vi "Config.vi"(8 "error in (no error)":errorcluster, 10 "Setting":variant, 11 "KE65XX DMM in":refnum<class "Keithley 65XX DMM.lvclass">) -> (0 "error out":errorcluster, 3 "KE65XX DMM out":refnum<class "Keithley 65XX DMM.lvclass">)   [LabVIEW 2025, in "DMM.lvlib" / "Keithley 65XX DMM.lvclass"]
uses:
  Keithley 65XX DMM.lvclass
  C:/Users/Public/Documents/Sandia National Labs/TSS Plugin/CEF.lvlibp/Node/CEF_Node.lvclass
  C:/Working copy/TS Manager/Plugin/Engines/DMM/DMM Instrument/DMM Instrument.lvclass
  C:/Users/Public/Documents/Sandia National Labs/TSS Plugin/Abstract Engine.lvlibp/Abstract Instrument/Abstract Instrument.lvclass
  DMM configuration/DMM configuration.lvclass
  Keithley 65XX DMM.lvclass/Keithley 65XX DMM.ctl
  DMM configuration/DMM configuration.lvclass/DMM configuration.ctl
  DMM Channel/DMM Channel.lvclass
  Users/Public/Documents/Sandia National Labs/TSS Plugin/Abstract Engine.lvlibp/Abstract Instrument/Channel.ctl
  Users/Public/Documents/Sandia National Labs/TSS Plugin/Abstract Engine.lvlibp/Abstract Instrument/Data Type.ctl
  Users/Public/Documents/Sandia National Labs/TSS Plugin/Abstract Engine.lvlibp/Channel configuration/Channel configuration.lvclass
  DMM configuration/Read DMM Setting.vi
  Users/Public/Documents/Sandia National Labs/TSS Plugin/CEF.lvlibp/Node/ReadChildren.vi
  Users/Public/Documents/Sandia National Labs/TSS Plugin/Abstract Engine.lvlibp/Channel configuration/Read Channel Setting.vi
  Users/Public/Documents/Sandia National Labs/TSS Plugin/CEF.lvlibp/Node/CEF_Node.lvclass
  Users/Public/Documents/Sandia National Labs/TSS Plugin/CEF.lvlibp/serializable configuration/CEF_serializable configuration.lvclass
  <instrlib>/Keithley DMM6500 DAQ6500 Series/Keithley DMM6500 DAQ6500 Series.lvlib
  Users/Public/Documents/Sandia National Labs/TSS Plugin/Abstract Engine.lvlibp/Abstract Instrument/Abstract Instrument.lvclass
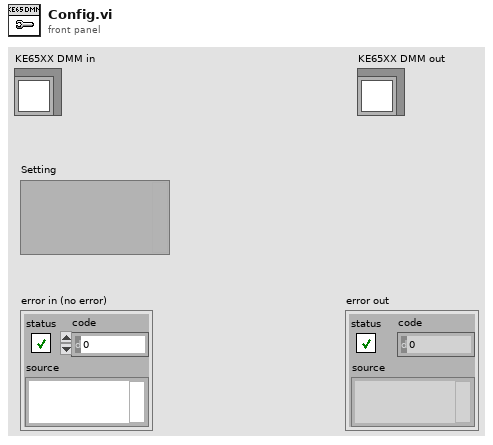
[diagram p1: front panel]
types:
  T1 = typedef "DMM.lvlib/DMM configuration.lvclass/DMM Setting.ctl" = cluster{"Function":string, "CurrentSource":string, "Resolution":string, "Range":dbl}
  T2 = typedef "Abstract Engine.lvlibp/Abstract Instrument.lvclass/Channel.ctl" = cluster{"Alias":string, "DataType":T3, "Unit":enum16{"---", "V", "A", "Ohm", "Hz", "uF", "degC", "deg"}, "Upper limit":dbl, "Lower limit":dbl, "Measurement":variant}
  T3 = typedef "Abstract Engine.lvlibp/Abstract Instrument.lvclass/Data Type.ctl" = string
  T4 = typedef "Abstract Engine.lvlibp/Channel configuration.lvclass/Default Channel.ctl" = cluster{"Address":string, "SW Alias":string, "Enabled":bool, "Type":string, "Description":string}
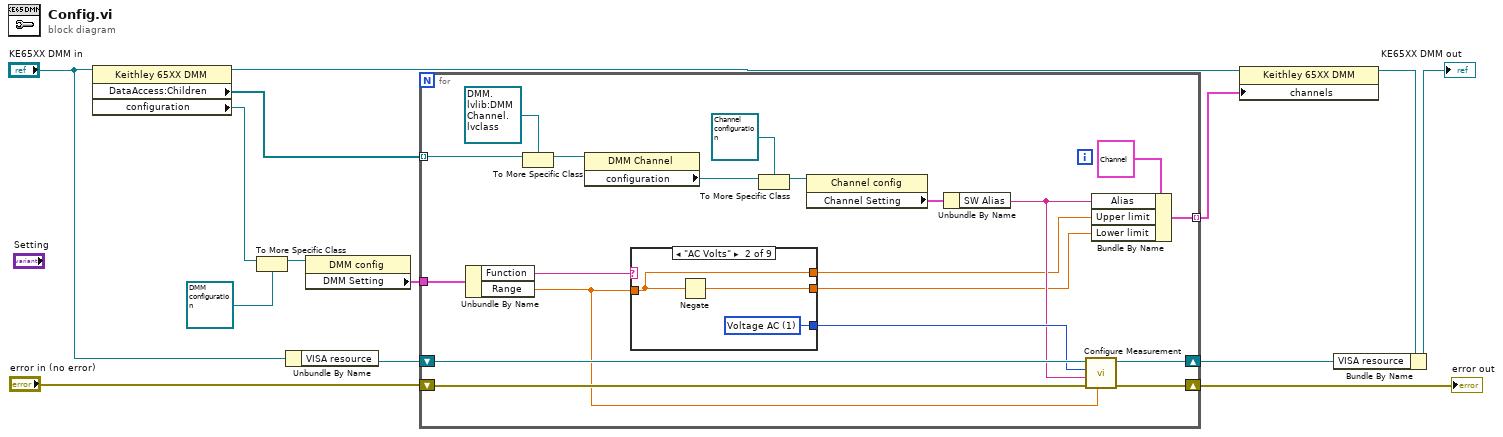
[diagram p0: block diagram]
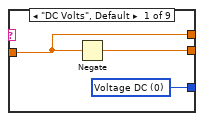
[diagram p2: hidden frame]
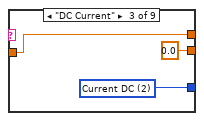
[diagram p3: hidden frame]
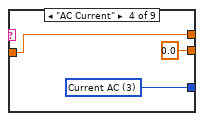
[diagram p4: hidden frame]
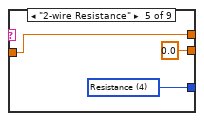
[diagram p5: hidden frame]
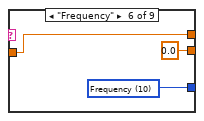
[diagram p6: hidden frame]
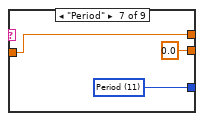
[diagram p7: hidden frame]
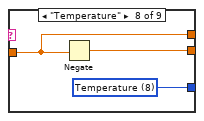
[diagram p8: hidden frame]
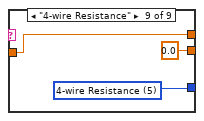
[diagram p9: hidden frame]
diagram:
  n1 = property class="Keithley 65XX DMM"(reference="KE65XX DMM in") -> (reference out=w11:refnum<class "Keithley 65XX DMM.lvclass">, "DataAccess:Children"=w8:refnum<data-value>[], "configuration"=w9:refnum<class "CEF_serializable configuration.lvclass">)  [unwired: 1 in, 1 out]
  n2 = To More Specific Class(target class=refnum<class "DMM configuration.lvclass"> refnum ("DMM.lvlib:DMM configuration.lvclass"), reference=w9) -> (specific class reference=w10:refnum<class "DMM configuration.lvclass">)  [unwired: 1 in, 1 out]
  n3 = Unbundle By Name("KE65XX DMM in") -> ("VISA resource"=w14:refnum<visa-resource-name>)
  n4 = property class="DMM config"(reference=w10) -> ("DMM Setting"=w5:T1)  [unwired: 1 in, 2 out]
  n5 = for {
    tunnel: w5 -> [w32]
    shift-right: [w33] -> w12
    shift-left: w14 -> [w34]
    tunnel: w8 -> [w29] mode=indexing
    shift-right: [w28] -> w7
    shift-left: "error in (no error)" -> [w27]
    tunnel: [w25] -> w1 mode=indexing
    n6 = Unbundle By Name(w32) -> ("Function"=w31:string, "Range"=w23:dbl)
    n7 = To More Specific Class(target class=refnum<data-value> refnum ("data value reference"), reference=w29) -> (specific class reference=w15:refnum<data-value>)  [unwired: 1 in, 1 out]
    n8 = property class="DMM Channel"(reference=w15) -> ("configuration"=w19:refnum<class "CEF_serializable configuration.lvclass">)  [unwired: 1 in, 2 out]
    n9 = case shown="\"AC Volts\"" w31 {
      tunnel: [w37 w40 w43 w46 w49 w52 w55 w58 w61] -> w30
      tunnel: w23 -> [w36 w39 w42 w45 w48 w51 w54 w57 w60]
      tunnel: [w36 w39 w42 w45 w48 w51 w54 w57 w60] -> w22
      tunnel: [w35 w38 0.0 0.0 0.0 0.0 0.0 w56 0.0] -> w21
      frame "DC Volts", Default {
        w37 = 0 items=[" Voltage DC", "Voltage AC", "Current DC", "Current AC", "Resistance", "4-wire Resistance", "Diode", "Capacitance", "Temperature", "Continuity", "Frequency", "Period", "Voltage Ratio"] ("Function (0: Voltage DC)")
        n10 = Negate(x=w36) -> (-x=w35:dbl)
      }
      frame "AC Volts" {
        w40 = 1 items=[" Voltage DC", "Voltage AC", "Current DC", "Current AC", "Resistance", "4-wire Resistance", "Diode", "Capacitance", "Temperature", "Continuity", "Frequency", "Period", "Voltage Ratio"] ("Function (0: Voltage DC)")
        n11 = Negate(x=w39) -> (-x=w38:dbl)
      }
      frame "DC Current" {
        w43 = 2 items=[" Voltage DC", "Voltage AC", "Current DC", "Current AC", "Resistance", "4-wire Resistance", "Diode", "Capacitance", "Temperature", "Continuity", "Frequency", "Period", "Voltage Ratio"] ("Function (0: Voltage DC)")
      }
      frame "AC Current" {
        w46 = 3 items=[" Voltage DC", "Voltage AC", "Current DC", "Current AC", "Resistance", "4-wire Resistance", "Diode", "Capacitance", "Temperature", "Continuity", "Frequency", "Period", "Voltage Ratio"] ("Function (0: Voltage DC)")
      }
      frame "2-wire Resistance" {
        w49 = 4 items=[" Voltage DC", "Voltage AC", "Current DC", "Current AC", "Resistance", "4-wire Resistance", "Diode", "Capacitance", "Temperature", "Continuity", "Frequency", "Period", "Voltage Ratio"] ("Function (0: Voltage DC)")
      }
      frame "Frequency" {
        w52 = 10 items=[" Voltage DC", "Voltage AC", "Current DC", "Current AC", "Resistance", "4-wire Resistance", "Diode", "Capacitance", "Temperature", "Continuity", "Frequency", "Period", "Voltage Ratio"] ("Function (0: Voltage DC)")
      }
      frame "Period" {
        w55 = 11 items=[" Voltage DC", "Voltage AC", "Current DC", "Current AC", "Resistance", "4-wire Resistance", "Diode", "Capacitance", "Temperature", "Continuity", "Frequency", "Period", "Voltage Ratio"] ("Function (0: Voltage DC)")
      }
      frame "Temperature" {
        w58 = 8 items=[" Voltage DC", "Voltage AC", "Current DC", "Current AC", "Resistance", "4-wire Resistance", "Diode", "Capacitance", "Temperature", "Continuity", "Frequency", "Period", "Voltage Ratio"] ("Function (0: Voltage DC)")
        n12 = Negate(x=w57) -> (-x=w56:dbl)
      }
      frame "4-wire Resistance" {
        w61 = 5 items=[" Voltage DC", "Voltage AC", "Current DC", "Current AC", "Resistance", "4-wire Resistance", "Diode", "Capacitance", "Temperature", "Continuity", "Frequency", "Period", "Voltage Ratio"] ("Function (0: Voltage DC)")
      }
    }
    n13 = To More Specific Class(target class=refnum<class "Channel configuration.lvclass"> refnum ("Abstract Engine.lvlibp:Channel config"), reference=w19) -> (specific class reference=w18:refnum<class "Channel configuration.lvclass">)  [unwired: 1 in, 1 out]
    n14 = property class="Channel config"(reference=w18) -> ("Channel Setting"=w17:T4)  [unwired: 1 in, 2 out]
    n15 = Unbundle By Name(w17) -> ("SW Alias"=w24:string)
    n16 = call <instrlib>:"Configure Measurement.vi"("Manual Range (1)"=w23, "error in (no error)"=w27, "Channel List(\"\")"=w24, "Function (0: Voltage DC)"=w30, "VISA resource name"=w34) -> ("error out"=w28:errorcluster, "VISA resource name out"=w33:refnum<visa-resource-name>)  [unwired: 5 in]
    n17 = Bundle By Name(cluster=T2 {"Alias"="ch0", "DataType"="Analog Input", "Unit"=enum."V", "Upper limit"=10.0, "Lower limit"=-10.0, "Measurement"=variant} ("Channel"), "Alias"=w24, "Upper limit"=w22, "Lower limit"=w21) -> (w25:T2)
  }
  "error out" <- w7
  n18 = property class="Keithley 65XX DMM"(reference=w11, "channels"=w1) -> (reference out=w2:refnum<class "Keithley 65XX DMM.lvclass">)  [unwired: 1 in, 1 out]
  n19 = Bundle By Name(cluster=w2, "VISA resource"=w12) -> (→"KE65XX DMM out":refnum<class "Keithley 65XX DMM.lvclass">)
